vi "Resistance_SMUResistanceTest.vi"(9 "DCPower_Parameters":T1[](array[typedef]) {"Source Delay" format="%.6p"; "Sense" items=["Local"=1008, "Remote"=1009]; "Aperture_time" format="%.6p"; "Current_range" format="%.6p"; "Current" format="%.6p"; "Voltage_range" format="%.6p"; "Voltage" format="%.6p"}, 10 "Pins":T2[](array[typedef]), 11 "Semiconductor Module Context":T3) -> (0 "error out":errorcluster)   [LabVIEW 2023, in "Resistance.lvlib"]
doc: "Measures the resistance using an SMU channel in order to perform simple Continuity Test"
uses:
  Resistance.lvlib
  <vilib>/NI_TestStand_SemiconductorModule/NI_TestStand_Semiconductor_Module.lvlibp/PinMap/General/SemiconductorModuleContext.ctl
  <vilib>/NI_TestStand_SemiconductorModule/NI_TestStand_Semiconductor_Module.lvlibp/PinMap/TagProvider/TSM_Pin.ctl
  ResourceHandling/TypeDefs/RH_DCPower_Parameters.ctl
  <vilib>/NI_TestStand_SemiconductorModule/NI_TestStand_Semiconductor_Module.lvlibp/PinMap/PinQueryContext/MultiplePinMultipleSessionQueryContext/MultiplePinMultipleSessionQueryContext.lvclass
  C:/Program Files/National Instruments/LabVIEW 2023/vi.lib/NI_TestStand_SemiconductorModule/NI_TestStand_Semiconductor_Module.lvlibp/PinMap/PinQueryContext/PinQueryContext.lvclass
  <vilib>/NI_TestStand_SemiconductorModule/NI_TestStand_Semiconductor_Module.lvlibp/PinMap/DC Power/PinsToNIDCPowerSessions.vi
  <vilib>/NI_TestStand_SemiconductorModule/NI_TestStand_Semiconductor_Module.lvlibp/PinMap/General/Publish/PublishDataDouble1D.vi
  ResourceHandling/ResourceHandling.lvlib
  <vilib>/NI_TestStand_SemiconductorModule/NI_TestStand_Semiconductor_Module.lvlibp
  C:/Program Files/National Instruments/LabVIEW 2023/vi.lib/NI_TestStand_SemiconductorModule/NI_TestStand_Semiconductor_Module.lvlibp/PinMap/PinQueryContext/MultipleSessionPinQueryContext.lvclass
  C:/Program Files/National Instruments/LabVIEW 2023/vi.lib/NI_TestStand_SemiconductorModule/NI_TestStand_Semiconductor_Module.lvlibp/PinMap/PinQueryContext/MultiplePinMultipleSessionQueryContext/MultiplePinMultipleSessionQueryContext.lvclass
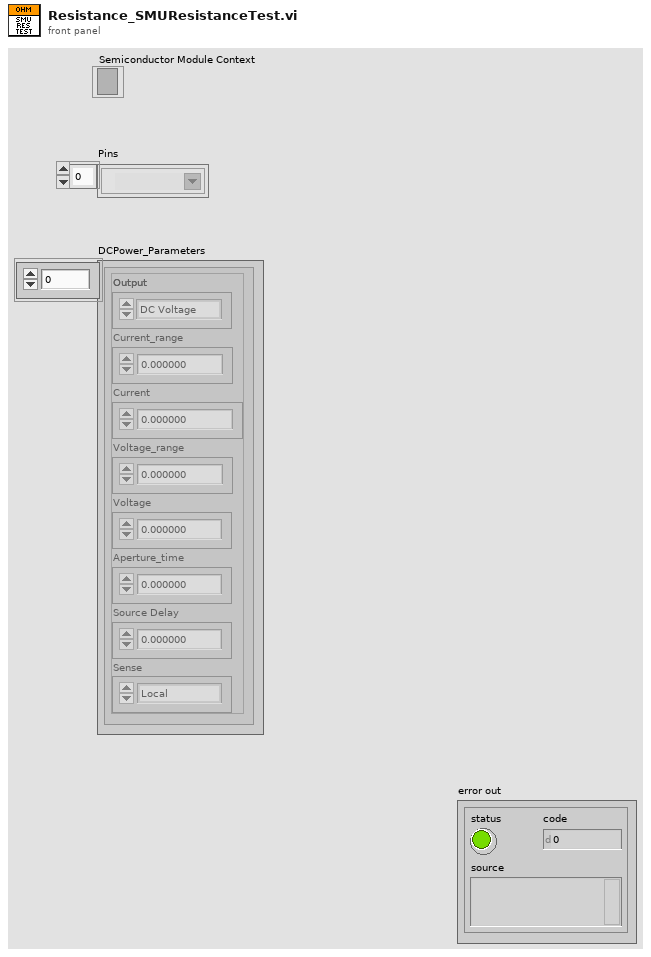
[diagram p1: front panel]
types:
  T1 = typedef "ResourceHandling.lvlib/RH_DCPower_Parameters.ctl" = cluster{"Output":enum16{"DC Voltage", "DC Current"}, "Current_range":dbl, "Current":dbl, "Voltage_range":dbl, "Voltage":dbl, "Aperture_time":dbl, "Source Delay":dbl, "Sense":i32}
  T2 = typedef "NI_TestStand_Semiconductor_Module.lvlibp/TSM_Pin.ctl" = tag
  T3 = typedef "NI_TestStand_Semiconductor_Module.lvlibp/SemiconductorModuleContext.ctl" = refnum<k7>
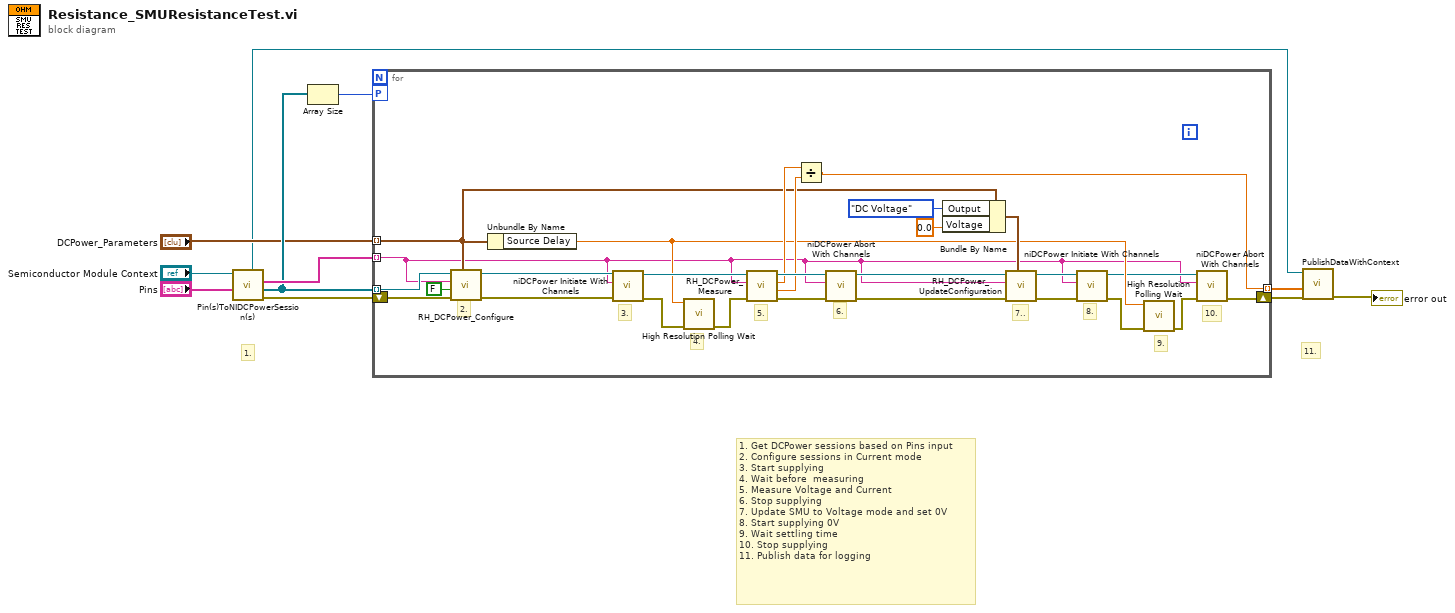
[diagram p0: block diagram]
diagram:
  # "11."
  # "1. Get DCPower sessions based on Pins input\n2. Configure sessions in Current mode\n3. Start supplying\n4. Wait before  measuring\n5. Measure Voltage and Current\n6. Stop supplying\n7. Update SMU to Voltage mode and set 0V\n8. Start supplying 0V\n9. Wait settling time\n10. Stop supplying\n11. Publish data for logging"
  # "1."
  n1 = call-poly <vilib>:"Pin(s)ToNIDCPowerSession(s).vi"("Pins"="Pins", "Semiconductor Module Context"="Semiconductor Module Context") -> ("error out"=w9:errorcluster, "Instrument Sessions"=w6:refnum<k15>[], "Channel Strings"=w8:string[], "Pin Query Context"=w2:refnum<class "MultiplePinMultipleSessionQueryContext.lvclass">)  [unwired: 5 in, 1 out]
  n2 = Array Size(array=w6) -> (size(s)=w7:i32)
  n3 = for {
    shift-right: [w13] -> w4
    shift-left: w9 -> [w38]
    tunnel: w8 -> [w14] mode=indexing
    tunnel: w6 -> [w37] mode=indexing
    workers-P: w7 -> [_]
    tunnel: "DCPower_Parameters" -> [w24] mode=indexing
    tunnel: [w12] -> w1 mode=indexing
    # "10."
    # "9."
    # "8."
    # "7.."
    # "6."
    # "5."
    # "4."
    # "3."
    # "2."
    n4 = call "RH_DCPower_Configure.vi"("DCPower_Parameters"=w24, "error in (no error)"=w38, "trigger out?"=FALSE, "channel name"=w14, "DCPower Session In"=w37) -> ("error out"=w34:errorcluster, "DCPower Session Out"=w35:refnum<k15>)  [unwired: 5 in]
    n5 = Unbundle By Name(w24) -> ("Source Delay"=w17:dbl)
    n6 = call <instrlib>:"niDCPower Initiate With Channels.vi"("error in (no error)"=w34, "channel name"=w14, "instrument handle"=w35) -> ("error out"=w33:errorcluster, "instrument handle out"=w32:refnum<k15>)  [unwired: 7 in]
    n7 = call <vilib>:"High Resolution Polling Wait.vi"("error in (no error)"=w33, "seconds to wait"=w17) -> ("error out"=w31:errorcluster)  [unwired: 9 in]
    n8 = call "RH_DCPower_Measure.vi"("error in (no error)"=w31, "channel name"=w14, "DCPower Session In"=w32) -> ("error out"=w30:errorcluster, "Current"=w27:dbl, "Voltage"=w28:dbl, "DCPower Session Out"=w29:refnum<k15>)  [unwired: 5 in]
    n9 = Divide(x=w28, y=w27) -> (x/y=w12:dbl)
    n10 = call <instrlib>:"niDCPower Abort With Channels.vi"("error in (no error)"=w30, "channel name"=w14, "instrument handle"=w29) -> ("error out"=w26:errorcluster, "instrument handle out"=w25:refnum<k15>)  [unwired: 7 in]
    n11 = Bundle By Name(cluster=w24, "Output"=enum16{"DC Voltage", "DC Current"}."DC Voltage", "Voltage"=0.0) -> (w23:T1)
    n12 = call "RH_DCPower_UpdateConfiguration.vi"("DCPower_Parameters"=w23, "error in (no error)"=w26, "channel name"=w14, "DCPower Session In"=w25) -> ("error out"=w20:errorcluster, "DCPower Session Out"=w19:refnum<k15>)  [unwired: 6 in]
    n13 = call <instrlib>:"niDCPower Initiate With Channels.vi"("error in (no error)"=w20, "channel name"=w14, "instrument handle"=w19) -> ("error out"=w18:errorcluster, "instrument handle out"=w15:refnum<k15>)  [unwired: 7 in]
    n14 = call <vilib>:"High Resolution Polling Wait.vi"("error in (no error)"=w18, "seconds to wait"=w17) -> ("error out"=w16:errorcluster)  [unwired: 9 in]
    n15 = call <instrlib>:"niDCPower Abort With Channels.vi"("error in (no error)"=w16, "channel name"=w14, "instrument handle"=w15) -> ("error out"=w13:errorcluster)  [unwired: 7 in, 1 out]
  }
  n16 = call-poly <vilib>:"PublishDataWithContext.vi"("error in (no error)"=w4, "Data In"=w1, "Pin Query Context"=w2) -> ("error out"=→"error out":errorcluster)  [unwired: 7 in, 1 out]
